vi "work1_Takeorder_and_Cook.vi"() -> ()   [LabVIEW 2026]
panel:
  in  "stop":bool
  out "Clients Served":i32
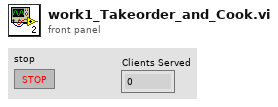
[diagram p1: front panel]
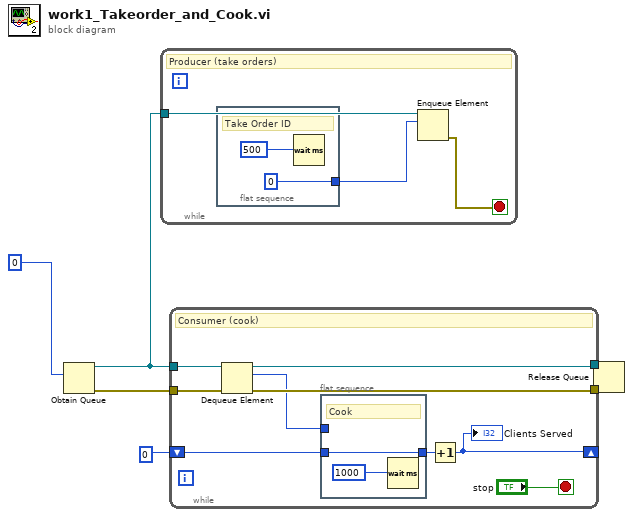
[diagram p0: block diagram]
diagram:
  n1 = Obtain Queue(element data type=0) -> (queue out=w5:refnum<queue>, error out=w4:errorcluster)  [unwired: 4 in, 1 out]
  n2 = while {
    tunnel: w5 -> [w8]
    stop <- w7 stop-if-true
    # "Producer (take orders)"
    n3 = flat-sequence {
      tunnel: [0] -> w9
      frame #0 {
        # "Take Order ID"
        n4 = Wait (ms)(milliseconds to wait=500) -> ()  [unwired: 1 out]
      }
    }
    n5 = Enqueue Element(queue=w8, element=w9) -> (error out=w7:errorcluster)  [unwired: 2 in, 2 out]
  }
  n6 = while {
    tunnel: w5 -> [w20]
    tunnel: w4 -> [w19]
    tunnel: [w18] -> w3
    tunnel: [w17] -> w2
    shift-right: [w14] -> _
    shift-left: 0 -> [w12]
    stop <- "stop" stop-if-true
    # "Consumer (cook)"
    n7 = Dequeue Element(queue=w20, error in (no error)=w19) -> (queue out=w17:refnum<queue>, element=w15:i32, error out=w18:errorcluster)  [unwired: 1 in, 1 out]
    n8 = flat-sequence {
      tunnel: w15 -> [_]
      tunnel: [w21] -> w13
      tunnel: w12 -> [w21]
      frame #0 {
        # "Cook"
        n9 = Wait (ms)(milliseconds to wait=1000) -> ()  [unwired: 1 out]
      }
    }
    n10 = Increment(x=w13) -> (x+1=w14:i32)
    "Clients Served" <- w14
  }
  n11 = Release Queue(queue=w2, error in (no error)=w3) -> ()  [unwired: 1 in, 3 out]
